vi "QueryFirst.vi"(6 "commandTimeout in":i32=-1, 7 "CommandType":i32(ring)=-1 items=["Text"=1, "StoredProcedure"=4, "TableDirect"=512], 8 "error in (no error)":errorcluster, 9 "DynamicParameters in":refnum<class "DynamicParameters.lvclass">, 10 "sql":string, 11 "PGJDPMapper in":refnum<class "Mapper.lvclass">) -> (0 "error out":errorcluster, 2 "Value":variant, 3 "PGJDPMapper out":refnum<class "Mapper.lvclass">)   [LabVIEW 2020, in "ORM_sqlite_jdp.lvlib" / "Mapper.lvclass"]
uses:
  Mapper.lvclass
  C:/Program Files/National Instruments/LabVIEW 2020/vi.lib/Viviota/shared/ORM.lvlibp/SqlMapper/SqlMapper.lvclass
  <vilib>/Viviota/shared/ORM.lvlibp/DynamicParameters/DynamicParameters.lvclass
  dbc/DBC.lvclass
  PGJDPParameter/Parameter.lvclass
  C:/Program Files/National Instruments/LabVIEW 2020/vi.lib/Viviota/shared/ORM.lvlibp/DynamicParameters/DynamicParameters.lvclass
  <vilib>/drjdpowell/SQLite Library/SQL Statement/SQL Statement.lvclass/SQL Statement.ctl
  <vilib>/drjdpowell/SQLite Library/SQL Statement/Next Bind (name).vi
  <vilib>/drjdpowell/SQLite Library/SQL Statement/Next Bind.vi
  <vilib>/drjdpowell/SQLite Library/SQL Statement/Step.vi
  <vilib>/Viviota/shared/ORM.lvlibp/SqlMapper/Read DbConnection.vi
  dbc/Read Connection.vi
  <vilib>/Viviota/shared/ORM.lvlibp/DynamicParameters/Read ParameterNames.vi
  <vilib>/Viviota/shared/ORM.lvlibp/DynamicParameters/Read ParameterValues.vi
  <vilib>/drjdpowell/SQLite Library/SQL Statement/Bind Parameters.vi
  <vilib>/drjdpowell/SQLite Library/SQL Statement/Error Message.vi
  <vilib>/Viviota/shared/ORM.lvlibp/DbConnection/DbConnection.lvclass
  <vilib>/drjdpowell/SQLite Library/SQL Connection/Connection.lvclass
  PGJDPResult/Result.lvclass
  <vilib>/drjdpowell/SQLite Library/SQL Statement/SQL Statement.lvclass
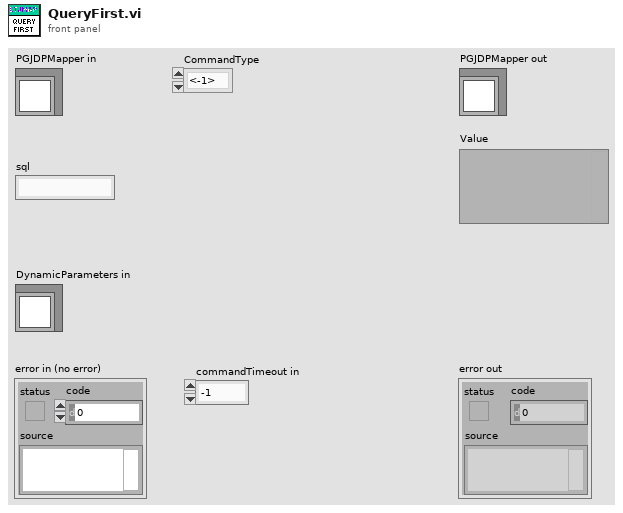
[diagram p1: front panel]
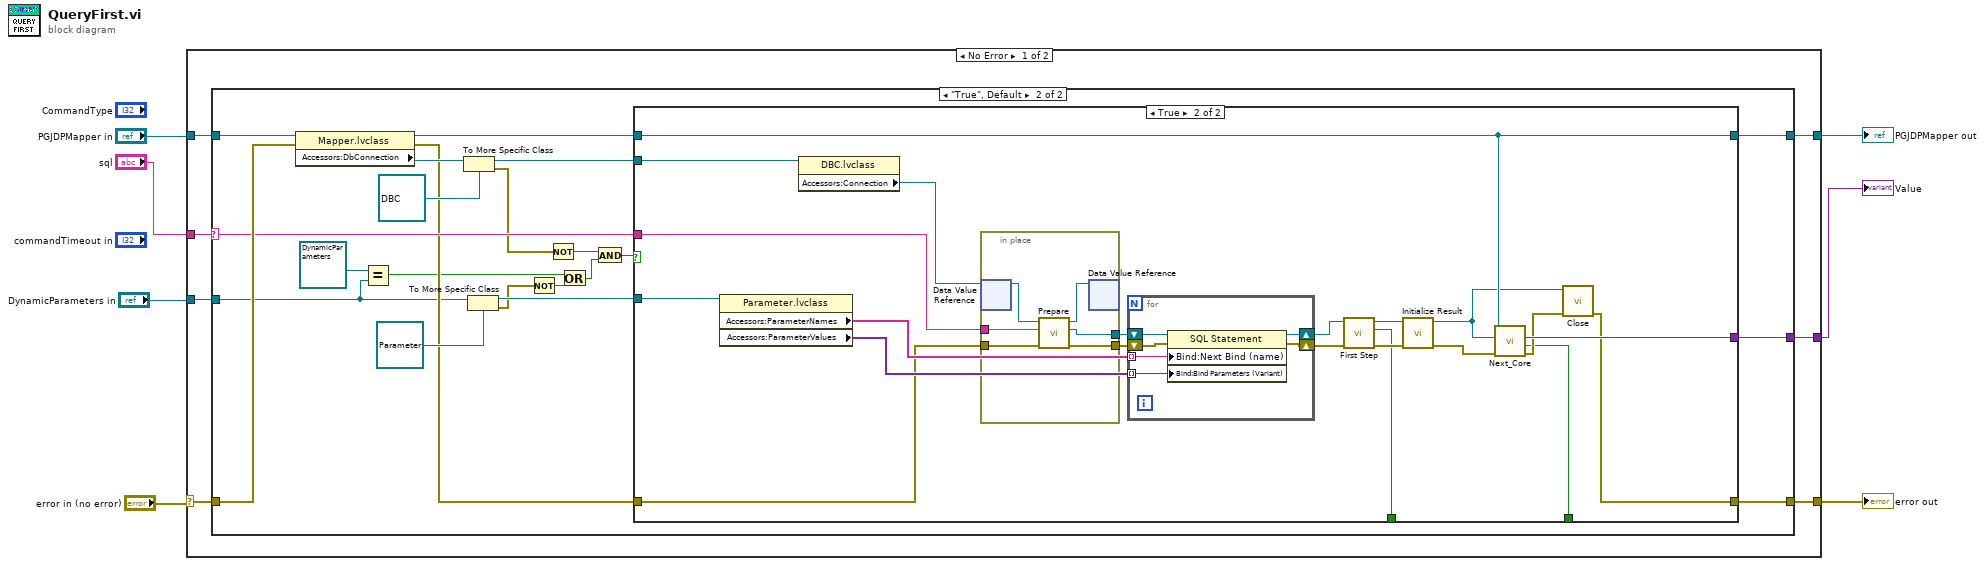
[diagram p0: block diagram]
diagram:
  n1 = case shown="No Error" "error in (no error)" {
    selector: "error in (no error)" -> [w12 w75]
    tunnel: "PGJDPMapper in" -> [w14 w74]
    tunnel: [w13 w74] -> w6
    tunnel: [w11 w75] -> w3
    tunnel: "sql" -> [w10 _]
    tunnel: "DynamicParameters in" -> [w9 _]
    tunnel: [w8 _] -> w2
    frame No Error {
      n2 = case shown="\"True\", Default" w10 {
        selector: w10 -> [_ w32]
        tunnel: w14 -> [w16 w38]
        tunnel: [w16 w26] -> w13
        tunnel: w12 -> [w15 w37]
        tunnel: [w15 w29] -> w11
        tunnel: w9 -> [_ w17]
        tunnel: [_ w28] -> w8
        frame "" {
        }
        frame "True", Default {
          n3 = property class="Mapper.lvclass"(reference=w38, error in=w37) -> (reference out=w27:refnum<class "Mapper.lvclass">, error out=w30:errorcluster, "Accessors:DbConnection"=w36:refnum<class "DbConnection.lvclass">)
          n4 = Equal?(x=refnum<class "DynamicParameters.lvclass"> refnum ("DynamicParameters"), y=w17) -> (x = y?=w23:bool)
          n5 = To More Specific Class(target class=refnum<class "DBC.lvclass"> refnum ("ORM_pgsql_jdp.lvlib:DBC.lvclass"), reference=w36) -> (specific class reference=w31:refnum<class "DBC.lvclass">, error out=w20:errorcluster)  [unwired: 1 in]
          n6 = To More Specific Class(target class=refnum<class "Parameter.lvclass"> refnum ("ORM_pgsql_jdp.lvlib:PGJDPParameter.lvclass"), reference=w17) -> (specific class reference=w33:refnum<class "Parameter.lvclass">, error out=w19:errorcluster)  [unwired: 1 in]
          n7 = Not(x=w19) -> (.not. x?=w24:bool)
          n8 = Not(x=w20) -> (.not. x?=w21:bool)
          n9 = Or(x=w23, y=w24) -> (x .or. y?=w22:bool)
          n10 = And(x=w21, y=w22) -> (x .and. y?=w18:bool)
          n11 = case shown="True" w18 {
            tunnel: w33 -> [_ w49]
            tunnel: w32 -> [_ w50]
            tunnel: w31 -> [_ w51]
            tunnel: w30 -> [w40 w48]
            tunnel: [w40 w43] -> w29
            tunnel: [_ w61] -> w28
            tunnel: w27 -> [w39 w46]
            tunnel: [w39 w46] -> w26
            tunnel: [_ w42] -> _
            tunnel: [_ w41] -> _
            frame False {
            }
            frame True {
              n12 = property class="Parameter.lvclass"(reference=w49) -> ("Accessors:ParameterNames"=w58:string[], "Accessors:ParameterValues"=w57:variant[])  [unwired: 1 in, 2 out]
              n13 = property class="DBC.lvclass"(reference=w51) -> ("Accessors:Connection"=w54:refnum<data-value>)  [unwired: 1 in, 2 out]
              n14 = in-place {
                in-place-border: w48 -> [w67]
                in-place-border: w50 -> [w66]
                in-place-border: [w65] -> w60
                in-place-border: [w64] -> w59
                n15 = in-place-dvr #1(w54) -> (w63:refnum<class "Connection.lvclass">)  [unwired: 1 out]
                n16 = call <vilib>:"Prepare.vi"("error in (no error)"=w67, "SQL"=w66, "SQLite Connection in"=w63) -> ("error out"=w65:errorcluster, "SQL Statement"=w64:refnum<class "SQL Statement.lvclass">, "SQLite Connection"=w62:refnum<class "Connection.lvclass">)  [unwired: 4 in, 2 out]
                n17 = in-place-dvr #1(w62) -> ()  [unwired: 2 out]
              }
              n18 = for {
                tunnel: w58 -> [w71] mode=indexing
                tunnel: w57 -> [w70] mode=indexing
                shift-right: [w69] -> w56
                shift-left: w59 -> [w72]
                shift-right: [w68] -> w55
                shift-left: w60 -> [w73]
                n19 = property class="SQL Statement"(reference=w72, error in=w73, "Bind:Next Bind (name)"=w71, "Bind:Bind Parameters (Variant)"=w70) -> (reference out=w69:refnum<class "SQL Statement.lvclass">, error out=w68:errorcluster)
              }
              n20 = call <vilib>:"First Step.vi"("error in (no error)"=w55, "SQL Statement in"=w56) -> ("error out"=w52:errorcluster, "Row returned"=w42:bool, "SQL Statement"=w53:refnum<class "SQL Statement.lvclass">)  [unwired: 7 in]
              n21 = call "Initialize Result.vi"("error in (no error)"=w52, "SQL Statement"=w53) -> ("error out"=w47:errorcluster, "PGJDPResult out"=w44:refnum<class "Result.lvclass">)  [unwired: 8 in]
              n22 = call-dynamic "Next_Core.vi"("error in (no error)"=w47, "PGJDPResult in"=w44, "SqlMapper in"=w46) -> ("error out"=w45:errorcluster, "Found"=w41:bool, "Row as Variant"=w61:variant)  [unwired: 5 in, 1 out]
              n23 = call-dynamic "Close.vi"("error in (no error)"=w45, "PGJDPResult in"=w44) -> ("error out"=w43:errorcluster)  [unwired: 9 in]
            }
          }
        }
      }
    }
    frame Error {
    }
  }
  "error out" <- w3
  "PGJDPMapper out" <- w6
  "Value" <- w2
